vi "VIH Project - Get Effective File Rule - Inherit.vi"(7 "Ignore Control Rules (F)":bool, 8 "PolyVI Instance VI":bool, 9 "File Type":T1, 10 "File Rule":T2, 11 "Parent Group Rule":T10) -> (2 "Effective File Rule":T2)   [LabVIEW 2014]
doc: "::: VI Helpeks :::\nCopyright (c) 2000-2026 Konstantin Shifershteyn. All rights reserved."
uses:
  _VIH HelpGen.llb/VIH HelpGen Typedef - Cluster - File Rule.ctl
  _VIH HelpGen.llb/VIH HelpGen Typedef - Enum - Default,Enable,Disable.ctl
  _VIH HelpGen.llb/VIH HelpGen Typedef - Cluster - File Rule - Source Paths.ctl
  _VIH HelpGen.llb/VIH HelpGen Typedef - Cluster - File Rule - Target Paths.ctl
  _VIH HelpGen.llb/VIH HelpGen Typedef - Enum - Description Mode.ctl
  _VIH HelpGen.llb/VIH HelpGen Typedef - Cluster - Control Rule.ctl
  _VIH HelpGen.llb/VIH HelpGen Typedef - Cluster - Enum Value Info.ctl
  _VIH HelpGen.llb/VIH HelpGen Typedef - Cluster - Group Rule - Flags.ctl
  _VIH HelpGen.llb/VIH HelpGen Typedef - Cluster - Group Rule.ctl
  _VIH HelpGen.llb/VIH HelpGen Typedef - Cluster - Group Rule - Source Paths.ctl
  _VIH HelpGen.llb/VIH HelpGen Typedef - Cluster - Group Rule - Target Paths.ctl
  _VIH HelpGen - Palette.llb/VIH HelpGen Typedef - Palette - Item Type Enum.ctl
panel:
  # "VI Helpeks\nCopyright (c) 2012-2026 Konstantin Shifershteyn"
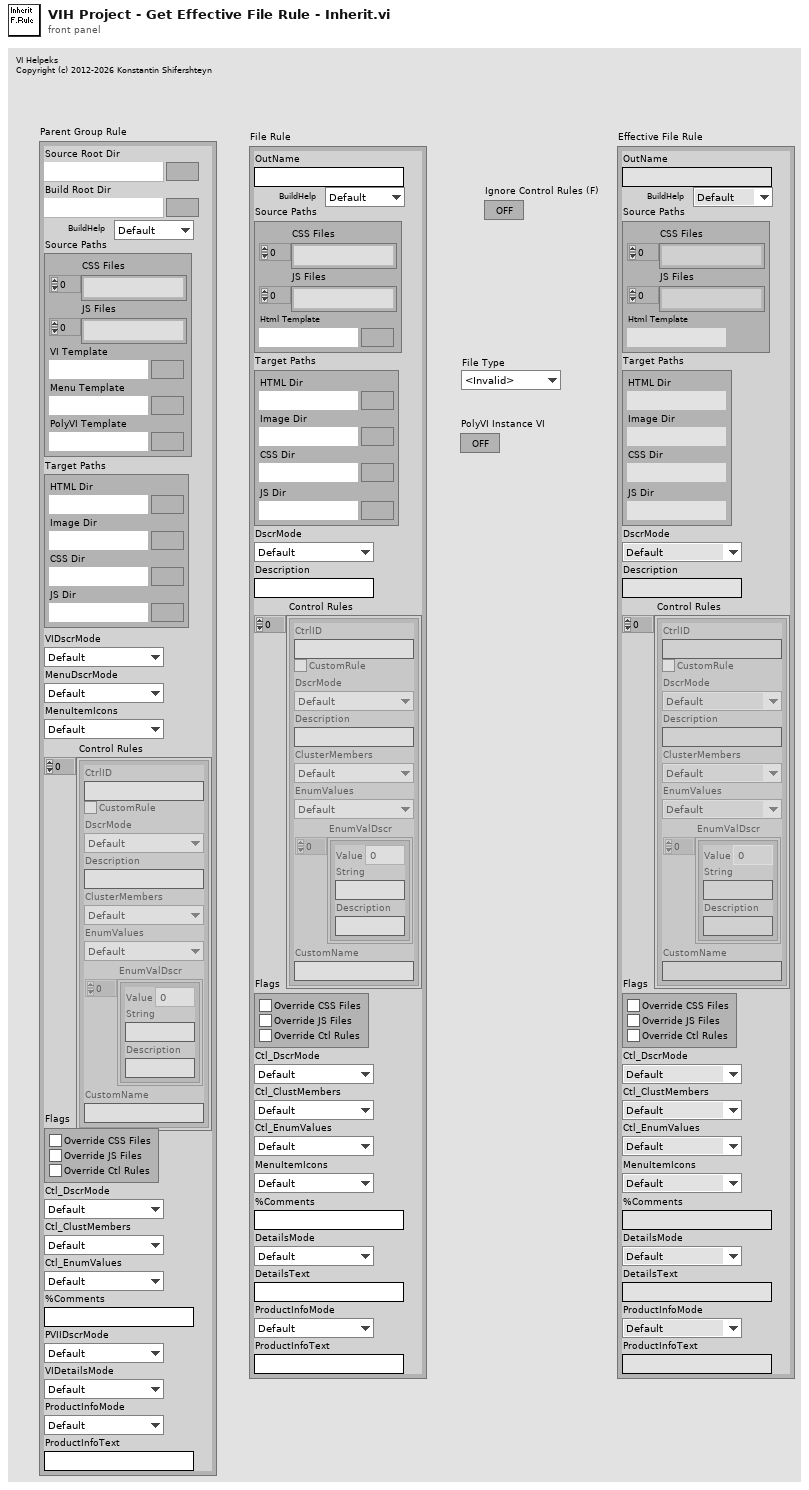
[diagram p1: front panel]
types:
  T1 = typedef "VIH HelpGen Typedef - Palette - Item Type Enum.ctl" = enum32{"<Invalid>", "<unknown>", "VI", "Menu", "LV Func", "Express VI", "Poly VI", "CTL", "HTML"}
  T2 = typedef "VIH HelpGen Typedef - Cluster - File Rule.ctl" = cluster{"OutName":string, "BuildHelp":T3, "Source Paths":T4, "Target Paths":T5, "DscrMode":T6, "Description":string, "Control Rules":T7[], "Flags":T9, "Ctl_DscrMode":T6, "Ctl_ClustMembers":T3, "Ctl_EnumValues":T3, "MenuItemIcons":T3, "%Comments":string, "DetailsMode":T6, "DetailsText":string, "ProductInfoMode":T3, "ProductInfoText":string}
  T3 = typedef "VIH HelpGen Typedef - Enum - Default,Enable,Disable.ctl" = enum16{"Default", "Enable", "Disable"}
  T4 = typedef "VIH HelpGen Typedef - Cluster - File Rule - Source Paths.ctl" = cluster{"CSS Files":path[], "JS Files":path[], "Html Template":path}
  T5 = typedef "VIH HelpGen Typedef - Cluster - File Rule - Target Paths.ctl" = cluster{"HTML Dir":path, "Image Dir":path, "CSS Dir":path, "JS Dir":path}
  T6 = typedef "VIH HelpGen Typedef - Enum - Description Mode.ctl" = enum16{"Default", "Description", "Description1", "Description2", "Custom", "None"}
  T7 = typedef "VIH HelpGen Typedef - Cluster - Control Rule.ctl" = cluster{"CtrlID":string, "CustomRule":bool, "DscrMode":T6, "Description":string, "ClusterMembers":T3, "EnumValues":T3, "EnumValDscr":T8[], "CustomName":string}
  T8 = typedef "VIH HelpGen Typedef - Cluster - Enum Value Info.ctl" = cluster{"Value":ext, "String":string, "Description":string}
  T9 = typedef "VIH HelpGen Typedef - Cluster - Group Rule - Flags.ctl" = cluster{"Override CSS Files":bool, "Override JS Files":bool, "Override Ctl Rules":bool}
  T10 = typedef "VIH HelpGen Typedef - Cluster - Group Rule.ctl" = cluster{"Source Root Dir":path, "Build Root Dir":path, "BuildHelp":T3, "Source Paths":T11, "Target Paths":T12, "VIDscrMode":T6, "MenuDscrMode":T6, "MenuItemIcons":T3, "Control Rules":T7[], "Flags":T9, "Ctl_DscrMode":T6, "Ctl_ClustMembers":T3, "Ctl_EnumValues":T3, "%Comments":string, "PVIIDscrMode":T6, "VIDetailsMode":T6, "ProductInfoMode":T3, "ProductInfoText":string}
  T11 = typedef "VIH HelpGen Typedef - Cluster - Group Rule - Source Paths.ctl" = cluster{"CSS Files":path[], "JS Files":path[], "VI Template":path, "Menu Template":path, "PolyVI Template":path}
  T12 = typedef "VIH HelpGen Typedef - Cluster - Group Rule - Target Paths.ctl" = cluster{"HTML Dir":path, "Image Dir":path, "CSS Dir":path, "JS Dir":path}
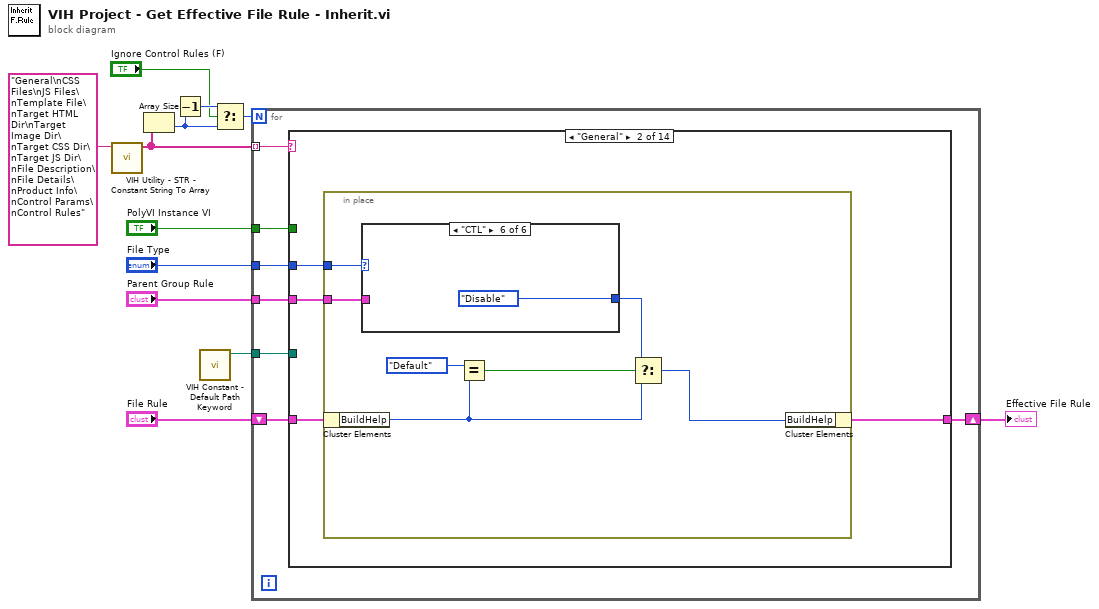
[diagram p0: block diagram]
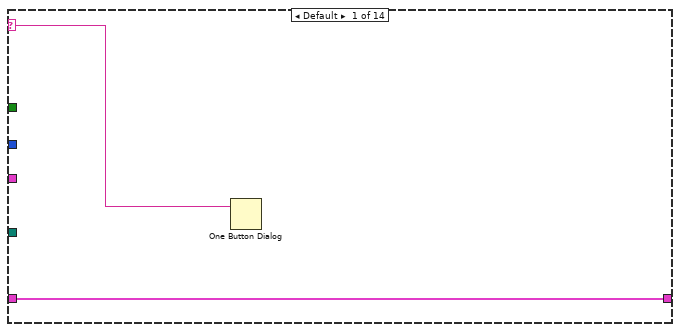
[diagram p2: hidden frame]
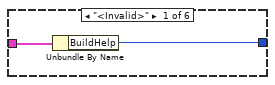
[diagram p3: hidden frame]
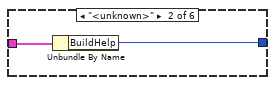
[diagram p4: hidden frame]
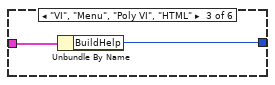
[diagram p5: hidden frame]
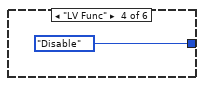
[diagram p6: hidden frame]
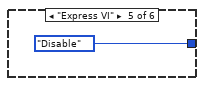
[diagram p7: hidden frame]
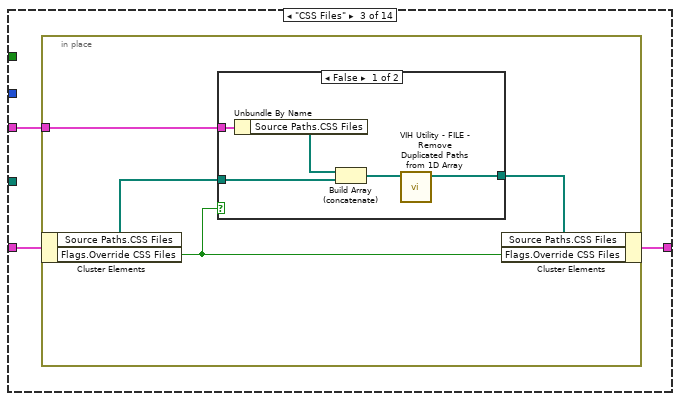
[diagram p8: hidden frame]
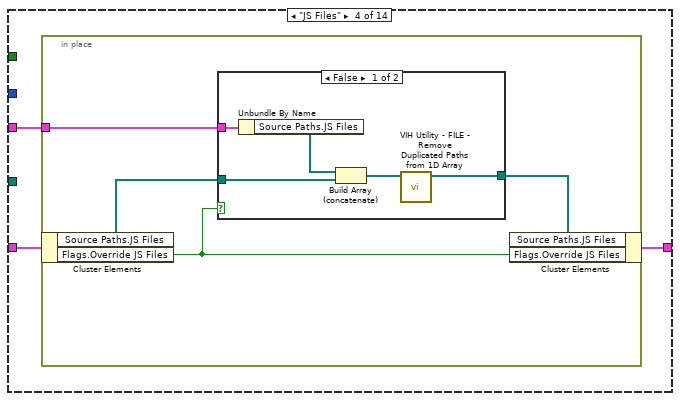
[diagram p10: hidden frame]
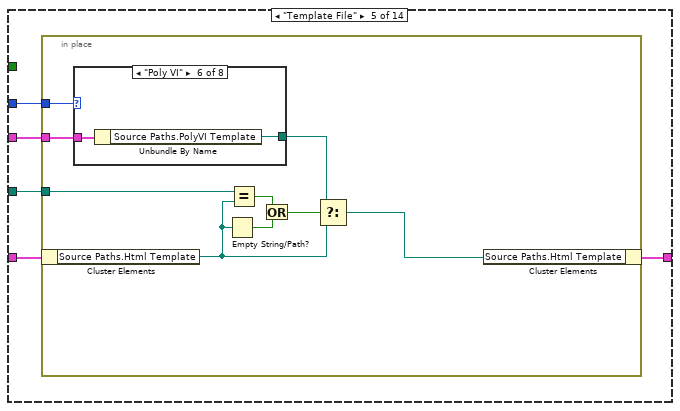
[diagram p12: hidden frame]
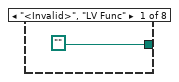
[diagram p13: hidden frame]
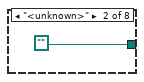
[diagram p14: hidden frame]
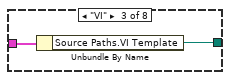
[diagram p15: hidden frame]
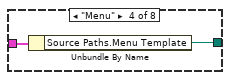
[diagram p16: hidden frame]
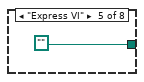
[diagram p17: hidden frame]
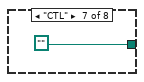
[diagram p18: hidden frame]
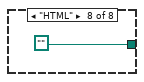
[diagram p19: hidden frame]
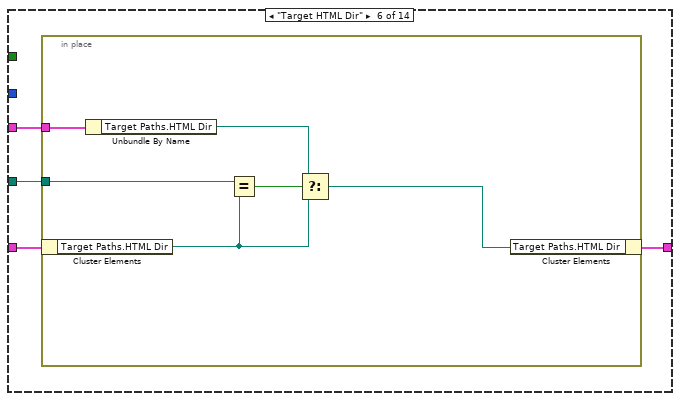
[diagram p20: hidden frame]
diagram:
  n1 = call "VIH Utility - STR - Constant String To Array.vi"("String in"="General\nCSS Files\nJS Files\nTemplate File\nTarget HTML Dir\nTarget Image Dir\nTarget CSS Dir\nTarget JS Dir\nFile Description\nFile Details\nProduct Info\nControl Params\nControl Rules") -> ("Array out"=w8:string[])  [unwired: 10 in]
  n2 = Array Size(array=w8) -> (size(s)=w6:i32)
  n3 = Decrement(x=w6) -> (x-1=w7:i32)
  n4 = call "VIH Constant - Default Path Keyword.vi"() -> ("<default> path"=w2:path)  [unwired: 11 in]
  n5 = Select(t=w7, s="Ignore Control Rules (F)", f=w6) -> (s? t:f=w4:i32)
  n6 = for {
    N: w4 -> [_]
    tunnel: w8 -> [w19] mode=indexing
    shift-right: [w18] -> w10
    shift-left: "File Rule" -> [w17]
    tunnel: "Parent Group Rule" -> [w16]
    tunnel: w2 -> [w15]
    tunnel: "File Type" -> [w14]
    tunnel: "PolyVI Instance VI" -> [w13]
    n7 = case shown="\"General\"" w19 {
      selector: w19 -> [w20 _ _ _ _ _ _ _ _ _ _ _ _ _]
      tunnel: [w21 w24 w43 w56 w71 w95 w105 w115 w125 w137 w174 w198 w238 w257] -> w18
      tunnel: w17 -> [w21 w25 w44 w57 w72 w96 w106 w116 w126 w138 w175 w199 w239 w258]
      tunnel: w16 -> [_ w23 w42 w55 w70 w94 w104 w114 w124 w136 w173 w197 w237 w256]
      tunnel: w15 -> [_ _ _ _ w69 w93 w103 w113 w123 w135 w172 w196 w236 _]
      tunnel: w14 -> [_ w22 _ _ w68 _ _ _ _ w134 w171 w195 _ _]
      tunnel: w13 -> [_ _ _ _ _ _ _ _ _ w133 w170 w194 _ _]
      frame Default {
        n8 = One Button Dialog(message=w20) -> ()  [unwired: 1 in, 1 out]
      }
      frame "General" {
        n9 = in-place {
          in-place-border: w23 -> [w32]
          in-place-border: w22 -> [w26]
          n10 = in-place-cluster #1(w25) -> ("BuildHelp"=w28:T3)
          n11 = case shown="\"CTL\"" w26 {
            tunnel: w32 -> [w34 w36 w38 _ _ _]
            tunnel: [w33 w35 w37 VIH_HelpGen_Typedef_-_Enum_-_Default,Enable,Disable."Disable" ("BuildHelp") VIH_HelpGen_Typedef_-_Enum_-_Default,Enable,Disable."Disable" ("BuildHelp") VIH_HelpGen_Typedef_-_Enum_-_Default,Enable,Disable."Disable" ("BuildHelp")] -> w29
            frame "<Invalid>" {
              n12 = Unbundle By Name(w34) -> ("BuildHelp"=w33:T3)
            }
            frame "<unknown>" {
              n13 = Unbundle By Name(w36) -> ("BuildHelp"=w35:T3)
            }
            frame "VI", "Menu", "Poly VI", "HTML" {
              n14 = Unbundle By Name(w38) -> ("BuildHelp"=w37:T3)
            }
            frame "LV Func" {
            }
            frame "Express VI" {
            }
            frame "CTL" {
            }
          }
          n15 = Equal?(x=VIH_HelpGen_Typedef_-_Enum_-_Default,Enable,Disable."Default", y=w28) -> (x = y?=w30:bool)
          n16 = Select(t=w29, s=w30, f=w28) -> (s? t:f=w27:T3)
          n17 = in-place-cluster #1("BuildHelp"=w27) -> (w24:T2)
        }
      }
      frame "CSS Files" {
        n18 = in-place {
          in-place-border: w42 -> [w48]
          n19 = in-place-cluster #2(w44) -> ("Source Paths.CSS Files"=w46:path[], "Flags.Override CSS Files"=w45:bool)
          n20 = case shown="False" w45 {
            tunnel: w48 -> [w53 _]
            tunnel: [w49 w54] -> w47
            tunnel: w46 -> [w52 w54]
            frame False {
              n21 = Unbundle By Name(w53) -> ("Source Paths.CSS Files"=w51:path[])
              n22 = Build Array (concatenate)(w51, w52) -> (w50:path[])
              n23 = call "VIH Utility - FILE - Remove Duplicated Paths from 1D Array.vi"("Array in"=w50) -> ("Array out"=w49:path[])  [unwired: 9 in, 1 out]
            }
            frame True {
            }
          }
          n24 = in-place-cluster #2("Source Paths.CSS Files"=w47, "Flags.Override CSS Files"=w45) -> (w43:T2)
        }
      }
      frame "JS Files" {
        n25 = in-place {
          in-place-border: w55 -> [w61]
          n26 = in-place-cluster #3(w57) -> ("Source Paths.JS Files"=w59:path[], "Flags.Override JS Files"=w58:bool)
          n27 = case shown="False" w58 {
            tunnel: w61 -> [w66 _]
            tunnel: [w62 w67] -> w60
            tunnel: w59 -> [w65 w67]
            frame False {
              n28 = Unbundle By Name(w66) -> ("Source Paths.JS Files"=w64:path[])
              n29 = Build Array (concatenate)(w64, w65) -> (w63:path[])
              n30 = call "VIH Utility - FILE - Remove Duplicated Paths from 1D Array.vi"("Array in"=w63) -> ("Array out"=w62:path[])  [unwired: 9 in, 1 out]
            }
            frame True {
            }
          }
          n31 = in-place-cluster #3("Source Paths.JS Files"=w60, "Flags.Override JS Files"=w58) -> (w56:T2)
        }
      }
      frame "Template File" {
        n32 = in-place {
          in-place-border: w70 -> [w81]
          in-place-border: w69 -> [w74]
          in-place-border: w68 -> [w73]
          n33 = in-place-cluster #4(w72) -> ("Source Paths.Html Template"=w76:path)
          n34 = case shown="\"Poly VI\"" w73 {
            tunnel: w81 -> [_ _ w85 w87 _ w90 _ _]
            tunnel: [path "" path "" w84 w86 path "" w89 path "" path ""] -> w77
            frame "<Invalid>", "LV Func" {
            }
            frame "<unknown>" {
            }
            frame "VI" {
              n35 = Unbundle By Name(w85) -> ("Source Paths.VI Template"=w84:path)
            }
            frame "Menu" {
              n36 = Unbundle By Name(w87) -> ("Source Paths.Menu Template"=w86:path)
            }
            frame "Express VI" {
            }
            frame "Poly VI" {
              n37 = Unbundle By Name(w90) -> ("Source Paths.PolyVI Template"=w89:path)
            }
            frame "CTL" {
            }
            frame "HTML" {
            }
          }
          n38 = Empty String/Path?(string/path=w76) -> (empty?=w79:bool)
          n39 = Equal?(x=w74, y=w76) -> (x = y?=w80:bool)
          n40 = Or(x=w80, y=w79) -> (x .or. y?=w78:bool)
          n41 = Select(t=w77, s=w78, f=w76) -> (s? t:f=w75:path)
          n42 = in-place-cluster #4("Source Paths.Html Template"=w75) -> (w71:T2)
        }
      }
      frame "Target HTML Dir" {
        n43 = in-place {
          in-place-border: w94 -> [w102]
          in-place-border: w93 -> [w98]
          n44 = in-place-cluster #5(w96) -> ("Target Paths.HTML Dir"=w100:path)
          n45 = Unbundle By Name(w102) -> ("Target Paths.HTML Dir"=w101:path)
          n46 = Equal?(x=w98, y=w100) -> (x = y?=w97:bool)
          n47 = Select(t=w101, s=w97, f=w100) -> (s? t:f=w99:path)
          n48 = in-place-cluster #5("Target Paths.HTML Dir"=w99) -> (w95:T2)
        }
      }
      frame "Target Image Dir" {
        n49 = in-place {
          in-place-border: w104 -> [w112]
          in-place-border: w103 -> [w108]
          n50 = in-place-cluster #6(w106) -> ("Target Paths.Image Dir"=w110:path)
          n51 = Unbundle By Name(w112) -> ("Target Paths.Image Dir"=w111:path)
          n52 = Equal?(x=w108, y=w110) -> (x = y?=w107:bool)
          n53 = Select(t=w111, s=w107, f=w110) -> (s? t:f=w109:path)
          n54 = in-place-cluster #6("Target Paths.Image Dir"=w109) -> (w105:T2)
        }
      }
      frame "Target CSS Dir" {
        n55 = in-place {
          in-place-border: w114 -> [w122]
          in-place-border: w113 -> [w118]
          n56 = in-place-cluster #7(w116) -> ("Target Paths.CSS Dir"=w120:path)
          n57 = Unbundle By Name(w122) -> ("Target Paths.CSS Dir"=w121:path)
          n58 = Equal?(x=w118, y=w120) -> (x = y?=w117:bool)
          n59 = Select(t=w121, s=w117, f=w120) -> (s? t:f=w119:path)
          n60 = in-place-cluster #7("Target Paths.CSS Dir"=w119) -> (w115:T2)
        }
      }
      frame "Target JS Dir" {
        n61 = in-place {
          in-place-border: w124 -> [w132]
          in-place-border: w123 -> [w128]
          n62 = in-place-cluster #8(w126) -> ("Target Paths.JS Dir"=w130:path)
          n63 = Unbundle By Name(w132) -> ("Target Paths.JS Dir"=w131:path)
          n64 = Equal?(x=w128, y=w130) -> (x = y?=w127:bool)
          n65 = Select(t=w131, s=w127, f=w130) -> (s? t:f=w129:path)
          n66 = in-place-cluster #8("Target Paths.JS Dir"=w129) -> (w125:T2)
        }
      }
      frame "File Description" {
        n67 = in-place {
          in-place-border: w136 -> [w151]
          in-place-border: w135 -> [_]
          in-place-border: w134 -> [w145]
          in-place-border: w133 -> [w139]
          n68 = in-place-cluster #9(w138) -> ("DscrMode"=w149:T6, "MenuItemIcons"=w143:T3)
          n69 = case shown="\"VI\"" w145 {
            tunnel: w151 -> [_ _ w161 w164 w167 _]
            tunnel: [VIH_HelpGen_Typedef_-_Enum_-_Description_Mode."Description" ("VIDscrMode") VIH_HelpGen_Typedef_-_Enum_-_Description_Mode."Description" ("VIDscrMode") w157 w163 w166 VIH_HelpGen_Typedef_-_Enum_-_Description_Mode."Description" ("VIDscrMode")] -> w150
            tunnel: [VIH_HelpGen_Typedef_-_Enum_-_Default,Enable,Disable."Disable" ("MenuItemIcons") VIH_HelpGen_Typedef_-_Enum_-_Default,Enable,Disable."Disable" ("MenuItemIcons") VIH_HelpGen_Typedef_-_Enum_-_Default,Enable,Disable."Disable" ("MenuItemIcons") w162 VIH_HelpGen_Typedef_-_Enum_-_Default,Enable,Disable."Disable" ("MenuItemIcons") VIH_HelpGen_Typedef_-_Enum_-_Default,Enable,Disable."Disable" ("MenuItemIcons")] -> w140
            tunnel: w139 -> [_ _ w156 _ _ _]
            frame "<Invalid>", "LV Func" {
            }
            frame "<unknown>" {
            }
            frame "VI" {
              n70 = Unbundle By Name(w161) -> ("PVIIDscrMode"=w159:T6, "VIDscrMode"=w158:T6)
              n71 = Select(t=w159, s=w156, f=w158) -> (s? t:f=w157:T6)
            }
            frame "Menu" {
              n72 = Unbundle By Name(w164) -> ("MenuDscrMode"=w163:T6, "MenuItemIcons"=w162:T3)
            }
            frame "Express VI".."CTL" {
              n73 = Unbundle By Name(w167) -> ("VIDscrMode"=w166:T6)
            }
            frame "HTML" {
            }
          }
          n74 = Equal?(x=VIH_HelpGen_Typedef_-_Enum_-_Description_Mode."Default", y=w149) -> (x = y?=w147:bool)
          n75 = Equal?(x=VIH_HelpGen_Typedef_-_Enum_-_Default,Enable,Disable."Default", y=w143) -> (x = y?=w144:bool)
          n76 = Select(t=w150, s=w147, f=w149) -> (s? t:f=w148:T6)
          n77 = Select(t=w140, s=w144, f=w143) -> (s? t:f=w141:T3)
          n78 = in-place-cluster #9("DscrMode"=w148, "MenuItemIcons"=w141) -> (w137:T2)
        }
      }
      frame "File Details" {
        n79 = in-place {
          in-place-border: w173 -> [w183]
          in-place-border: w172 -> [_]
          in-place-border: w171 -> [w177]
          in-place-border: w170 -> [w176]
          n80 = in-place-cluster #10(w175) -> ("DetailsMode"=w181:T6)
          n81 = case shown="\"Menu\"" w177 {
            tunnel: w183 -> [_ _ w190 _ _ _]
            tunnel: [VIH_HelpGen_Typedef_-_Enum_-_Description_Mode."None" ("VIDscrMode") VIH_HelpGen_Typedef_-_Enum_-_Description_Mode."None" ("VIDscrMode") w188 VIH_HelpGen_Typedef_-_Enum_-_Description_Mode."None" ("VIDetailsMode") VIH_HelpGen_Typedef_-_Enum_-_Description_Mode."None" ("VIDetailsMode") VIH_HelpGen_Typedef_-_Enum_-_Description_Mode."None" ("VIDetailsMode")] -> w182
            tunnel: w176 -> [_ _ w187 _ _ _]
            frame "<Invalid>", "LV Func" {
            }
            frame "<unknown>" {
            }
            frame "VI" {
              n82 = Unbundle By Name(w190) -> ("VIDetailsMode"=w189:T6)
              n83 = Select(t=VIH_HelpGen_Typedef_-_Enum_-_Description_Mode."None", s=w187, f=w189) -> (s? t:f=w188:T6)
            }
            frame "Menu" {
            }
            frame "Express VI".."CTL" {
            }
            frame "HTML" {
            }
          }
          n84 = Equal?(x=VIH_HelpGen_Typedef_-_Enum_-_Description_Mode."Default", y=w181) -> (x = y?=w179:bool)
          n85 = Select(t=w182, s=w179, f=w181) -> (s? t:f=w180:T6)
          n86 = in-place-cluster #10("DetailsMode"=w180) -> (w174:T2)
        }
      }
      frame "Product Info" {
        n87 = in-place {
          in-place-border: w197 -> [w210]
          in-place-border: w196 -> [_]
          in-place-border: w195 -> [w207]
          in-place-border: w194 -> [w206]
          n88 = in-place-cluster #11(w199) -> ("ProductInfoMode"=w209:T3, "ProductInfoText"=w203:string)
          n89 = case shown="\"VI\"" w207 {
            tunnel: w210 -> [_ _ w220 w223 _ w227 w229]
            tunnel: [VIH_HelpGen_Typedef_-_Enum_-_Default,Enable,Disable."Disable" VIH_HelpGen_Typedef_-_Enum_-_Default,Enable,Disable."Disable" w218 w222 VIH_HelpGen_Typedef_-_Enum_-_Default,Enable,Disable."Disable" w226 w230] -> w202
            tunnel: w206 -> [_ _ w215 _ _ _ _]
            tunnel: [_ _ w213 w221 _ w225 w228] -> w201
            frame "<Invalid>", "LV Func" {
            }
            frame "<unknown>" {
            }
            frame "VI" {
              n90 = Unbundle By Name(w220) -> ("ProductInfoMode"=w219:T3, "ProductInfoText"=w216:string)
              n91 = Select(t=VIH_HelpGen_Typedef_-_Enum_-_Default,Enable,Disable."Disable", s=w215, f=w219) -> (s? t:f=w218:T3)
              n92 = Select(t="", s=w215, f=w216) -> (s? t:f=w213:string)
            }
            frame "Menu" {
              n93 = Unbundle By Name(w223) -> ("ProductInfoMode"=w222:T3, "ProductInfoText"=w221:string)
            }
            frame "Express VI", "CTL" {
            }
            frame "Poly VI" {
              n94 = Unbundle By Name(w227) -> ("ProductInfoMode"=w226:T3, "ProductInfoText"=w225:string)
            }
            frame "HTML" {
              n95 = disable-structure shown="Enabled" {
                disable-tunnel: [VIH_HelpGen_Typedef_-_Enum_-_Default,Enable,Disable."Disable" w235] -> w230
                disable-tunnel: w229 -> [_ w234]
                disable-tunnel: ["" w233] -> w228
                frame Enabled {
                }
                frame Disabled {
                  n96 = Unbundle By Name(w234) -> ("ProductInfoMode"=w235:T3, "ProductInfoText"=w233:string)
                }
              }
            }
          }
          n97 = Equal?(x=VIH_HelpGen_Typedef_-_Enum_-_Default,Enable,Disable."Default", y=w209) -> (x = y?=w204:bool)
          n98 = Select(t=w202, s=w204, f=w209) -> (s? t:f=w208:T3)
          n99 = Select(t=w201, s=w204, f=w203) -> (s? t:f=w200:string)
          n100 = in-place-cluster #11("ProductInfoMode"=w208, "ProductInfoText"=w200) -> (w198:T2)
        }
      }
      frame "Control Params" {
        n101 = in-place {
          in-place-border: w237 -> [w255]
          in-place-border: w236 -> [_]
          n102 = in-place-cluster #12(w239) -> ("Ctl_DscrMode"=w253:T6, "Ctl_ClustMembers"=w247:T3, "Ctl_EnumValues"=w246:T3)
          n103 = Unbundle By Name(w255) -> ("Ctl_DscrMode"=w254:T6, "Ctl_ClustMembers"=w244:T3, "Ctl_EnumValues"=w243:T3)
          n104 = Equal?(x=VIH_HelpGen_Typedef_-_Enum_-_Description_Mode."Default", y=w253) -> (x = y?=w251:bool)
          n105 = Equal?(x=VIH_HelpGen_Typedef_-_Enum_-_Default,Enable,Disable."Default", y=w247) -> (x = y?=w249:bool)
          n106 = Equal?(x=VIH_HelpGen_Typedef_-_Enum_-_Default,Enable,Disable."Default", y=w246) -> (x = y?=w248:bool)
          n107 = Select(t=w254, s=w251, f=w253) -> (s? t:f=w252:T6)
          n108 = Select(t=w244, s=w249, f=w247) -> (s? t:f=w242:T3)
          n109 = Select(t=w243, s=w248, f=w246) -> (s? t:f=w241:T3)
          n110 = in-place-cluster #12("Ctl_DscrMode"=w252, "Ctl_ClustMembers"=w242, "Ctl_EnumValues"=w241) -> (w238:T2)
        }
      }
      frame "Control Rules" {
        n111 = in-place {
          in-place-border: w256 -> [w266]
          n112 = in-place-cluster #13(w258) -> ("Control Rules"=w265:T7[], "Flags.Override Ctl Rules"=w264:bool, "Ctl_DscrMode"=w261:T6, "Ctl_ClustMembers"=w260:T3, "Ctl_EnumValues"=w259:T3)
          n113 = case shown="False" w264 {
            tunnel: w266 -> [w272 _]
            tunnel: [w267 w273] -> w263
            tunnel: w265 -> [w270 w274]
            frame False {
              n114 = Unbundle By Name(w272) -> ("Control Rules"=w271:T7[])
              n115 = call "VIH Project - Control Rule - Filter Out Unused Rules.vi"("Control Rules"=w271) -> ("Control Rules out"=w268:T7[])  [unwired: 10 in]
              n116 = call "VIH Project - Control Rule - Filter Out Unused Rules.vi"("Control Rules"=w270) -> ("Control Rules out"=w269:T7[])  [unwired: 10 in]
              n117 = call "VIH Project - Control Rule - Merge Rule Arrays.vi"("Control Rules"=w269, "Parent Control Rules"=w268) -> ("Control Rules out"=w267:T7[])  [unwired: 9 in]
            }
            frame True {
              n118 = call "VIH Project - Control Rule - Filter Out Unused Rules.vi"("Control Rules"=w274) -> ("Control Rules out"=w273:T7[])  [unwired: 10 in]
            }
          }
          n119 = call "VIH Project - Control Rule - Apply Default.vi"("default EnumValues"=w259, "default ClusterMembers"=w260, "default DscrMode"=w261, "Control Rules"=w263) -> ("Control Rules out"=w262:T7[])  [unwired: 7 in]
          n120 = in-place-cluster #13("Control Rules"=w262, "Flags.Override Ctl Rules"=w264, "Ctl_DscrMode"=w261, "Ctl_ClustMembers"=w260, "Ctl_EnumValues"=w259) -> (w257:T2)
        }
      }
    }
  }
  "Effective File Rule" <- w10
